vi "GD Manipulation.vi"(10 "B Gate delay":dbl=0.0004112, 11 "A Gate Delay":dbl=0.00020533) -> ()   [LabVIEW 2024]
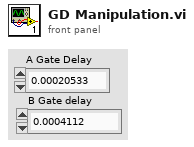
[diagram p1: front panel]
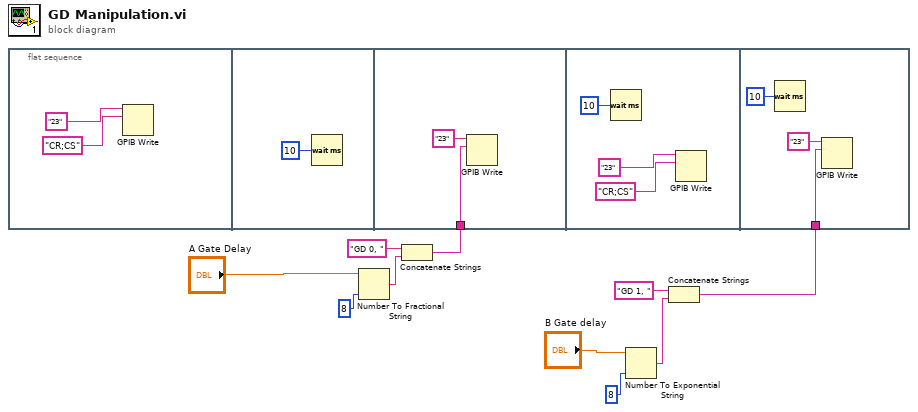
[diagram p0: block diagram]
diagram:
  n1 = flat-sequence {
    tunnel: w8 -> [w14]
    tunnel: w6 -> [w20]
    frame #0 {
      n2 = GPIB Write(0:"23" ("address string"), 1:"CR;CS" ("data")) -> ()  [unwired: 3 in, 2 out]
    }
    frame #1 {
      n3 = Wait (ms)(milliseconds to wait=u32 10) -> ()  [unwired: 1 out]
    }
    frame #2 {
      n4 = GPIB Write(0:"23" ("address string"), 1:w14) -> ()  [unwired: 3 in, 2 out]
    }
    frame #3 {
      n5 = Wait (ms)(milliseconds to wait=u32 10) -> ()  [unwired: 1 out]
      n6 = GPIB Write(0:"23" ("address string"), 1:"CR;CS" ("data")) -> ()  [unwired: 3 in, 2 out]
    }
    frame #4 {
      n7 = Wait (ms)(milliseconds to wait=u32 10) -> ()  [unwired: 1 out]
      n8 = GPIB Write(0:"23" ("address string"), 1:w20) -> ()  [unwired: 3 in, 2 out]
    }
  }
  n9 = Number To Fractional String(number="A Gate Delay", precision (6)=i16 8) -> (F-format string=w9:string)  [unwired: 2 in]
  n10 = Concatenate Strings("GD 0, " ("string"), w9) -> (w8:string)
  n11 = Number To Exponential String(number="B Gate delay", precision (6)=i16 8) -> (E-format string=w5:string)  [unwired: 2 in]
  n12 = Concatenate Strings("GD 1, " ("string"), w5) -> (w6:string)
